vi "ReceiveUDP.vi"() -> ()   [LabVIEW 2024]
panel:
  out "IP":string
  out "Arg6":u8
  out "Arg5":u8
  out "Arg7":u8
  out "Arg4":u8
  out "Arg3":u8
  out "Func2":u8
  out "Func1":u8
  out "Tail8":u8
  out "Head0":u8
  # "Receiver"
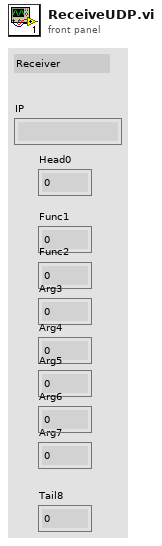
[diagram p1: front panel]
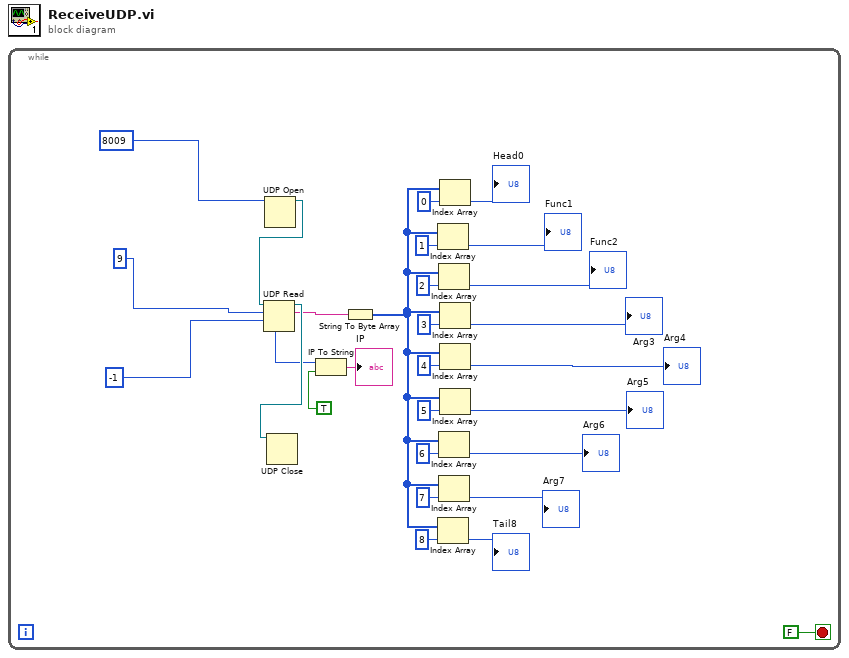
[diagram p0: block diagram]
diagram:
  n1 = while {
    stop <- FALSE stop-if-true
    n2 = UDP Open(11:u16 8009 ("port")) -> (port=w29:refnum<k16>)  [unwired: 4 in, 2 out]
    n3 = UDP Read(connection ID=w29, max size (548)=9, timeout ms (25000)=-1) -> (data out=w26:string, 3:w27:refnum<k16>, 6:w3:u32)  [unwired: 1 in, 2 out]
    n4 = UDP Close(connection ID=w27) -> ()  [unwired: 1 in, 2 out]
    n5 = IP To String(1:TRUE ("dot notation? (F)"), 2:w3) -> (0:→"IP":string)
    n6 = String To Byte Array(string=w26) -> (unsigned byte array=w16:u8[])
    n7 = Index Array(array=w16, index=1) -> (element=→"Func1":u8)
    n8 = Index Array(array=w16, index=8) -> (element=→"Tail8":u8)
    n9 = Index Array(array=w16, index=2) -> (element=→"Func2":u8)
    n10 = Index Array(array=w16, index=6) -> (element=→"Arg6":u8)
    n11 = Index Array(array=w16, index=7) -> (element=→"Arg7":u8)
    n12 = Index Array(array=w16, index=0) -> (element=→"Head0":u8)
    n13 = Index Array(array=w16, index=3) -> (element=→"Arg3":u8)
    n14 = Index Array(array=w16, index=4) -> (element=→"Arg4":u8)
    n15 = Index Array(array=w16, index=5) -> (element=→"Arg5":u8)
  }
